vi "Read Style.vi"(8 "error in (no error)":errorcluster, 11 "Splitter in":refnum<class "Splitter.lvclass">) -> (0 "error out":errorcluster, 2 "Style":T1 items=["Modern", "Classic", "System", "NXG"], 3 "Splitter out":refnum<class "Splitter.lvclass">)   [LabVIEW 2015, in "Splitter.lvclass"]
uses:
  Splitter.lvclass
  Typedefs/Splitter Style--Enum.ctl
  Splitter.lvclass/Splitter.ctl
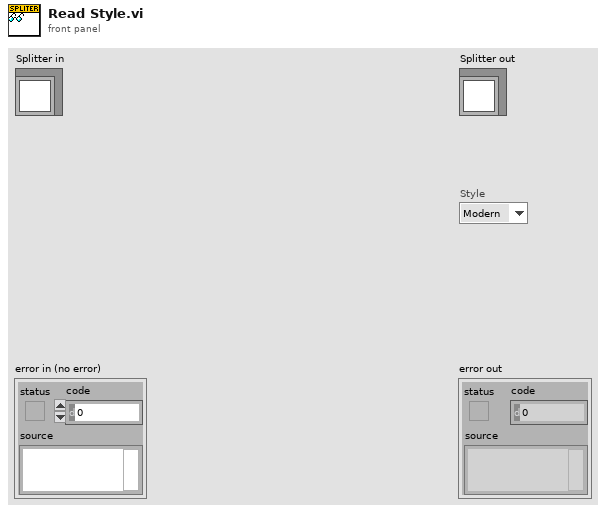
[diagram p1: front panel]
types:
  T1 = typedef "Splitter Style--Enum.ctl" = u16
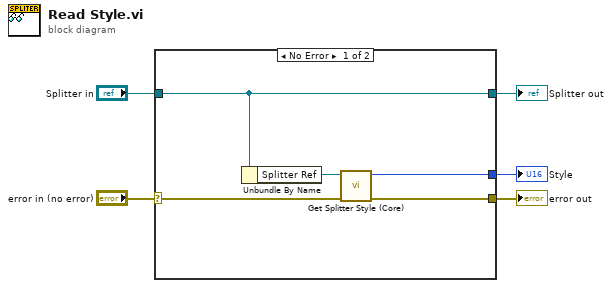
[diagram p0: block diagram]
diagram:
  n1 = case shown="No Error" "error in (no error)" {
    selector: "error in (no error)" -> [w9 w11]
    tunnel: [w8 w11] -> w4
    tunnel: [w10 w12] -> w2
    tunnel: "Splitter in" -> [w10 w12]
    tunnel: [w7 _] -> w1
    frame No Error {
      n2 = Unbundle By Name(w10) -> ("Splitter Ref"=w6:refnum<vi>)
      n3 = call "Get Splitter Style (Core).vi"("error in (no error)"=w9, "Splitter in"=w6) -> ("error out"=w8:errorcluster, "Style"=w7:T1)  [unwired: 6 in]
    }
    frame Error {
    }
  }
  "error out" <- w4
  "Splitter out" <- w2
  "Style" <- w1
